vi "G4SubTemplate_Singleton_6x8x6_Init.vi"(0 "reference in":refnum<class "G4SubTemplate_Singleton_6x8x6.lvclass"> caption="This control should only be used when\na sub class is inheriting this class", 5 "Error In":errorcluster) -> (14 "reference out":refnum<class "G4SubTemplate_Singleton_6x8x6.lvclass"> caption="This indicator should only be used when\na sub class is inheriting this class", 19 "Error Out":errorcluster)   [LabVIEW 2020, in "G4SubTemplate_Singleton_6x8x6.lvclass"]
uses:
  G4SubTemplate_Singleton_6x8x6.lvclass
  C:/VIT/GitHub/OpenGDS/resource/Framework/Providers/Open_GDS/ClassProviders/Provider_EndevoGOOP400/Templates/G4BaseTemplate_Singleton_6x8x6/G4BaseTemplate_Singleton_6x8x6.lvclass
  G4BaseTemplate_Singleton_6x8x6/G4BaseTemplate_Singleton_6x8x6.lvclass
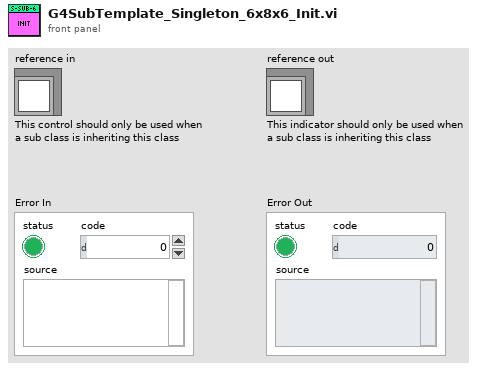
[diagram p1: front panel]
types:
  T1 = typedef "G4SubTemplate_Singleton_6x8x6.lvclass/ObjectAttributes.ctl" = cluster{"Attribute1":dbl}
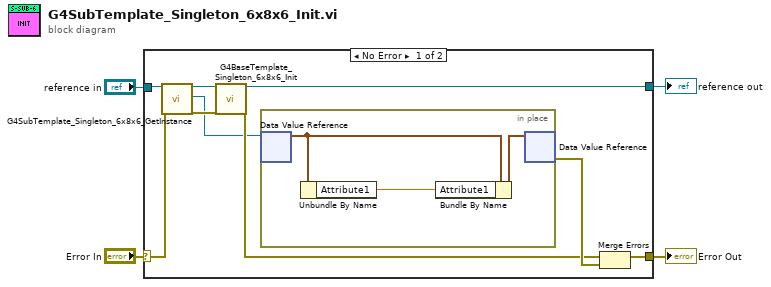
[diagram p0: block diagram]
diagram:
  n1 = case shown="No Error" "Error In" {
    selector: "Error In" -> [w10 w18]
    tunnel: [w12 w18] -> w3
    tunnel: "reference in" -> [w8 w17]
    tunnel: [w7 w17] -> w1
    frame No Error {
      n2 = call "G4SubTemplate_Singleton_6x8x6_GetInstance.vi"("reference in"=w8, "Error In"=w10) -> ("reference out"=w6:refnum<class "G4SubTemplate_Singleton_6x8x6.lvclass">, "DVRRefOut"=w5:refnum<data-value>, "Error Out"=w9:errorcluster)  [unwired: 13 in, 2 out]
      n3 = call "G4BaseTemplate_Singleton_6x8x6_Init.vi"("reference in"=w6, "Error In"=w9) -> ("reference out"=w7:refnum<class "G4SubTemplate_Singleton_6x8x6.lvclass">, "Error Out"=w11:errorcluster)  [unwired: 16 in]
      n4 = in-place {
        n5 = in-place-dvr #1(w5) -> (w15:T1)  [unwired: 1 out]
        n6 = Unbundle By Name(w15) -> ("Attribute1"=w14:dbl)
        n7 = Bundle By Name(cluster=w15, "Attribute1"=w14) -> (w16:T1)
        n8 = in-place-dvr #1(w16) -> (w13:errorcluster)  [unwired: 1 out]
      }
      n9 = Merge Errors(w11, w13) -> (w12:errorcluster)
    }
    frame Error {
    }
  }
  "Error Out" <- w3
  "reference out" <- w1
